vi "Network Close.vi"(8 "error in (no error)":errorcluster, 11 "Settings":T1={"UDP Receiver"=refnum, "UDP Sender"=refnum, "Valid Packet"=FALSE, "TCP"=refnum, "Network Settings"={"IP adress"="127.0.0.1", "RDB"={"Protocol"=enum."UDP", "Tx Port"=48270, "Rx Port"=10, "Buffer Size"=204800, "Timeout"=10}, "SCP"={"Protocol"=enum."TCP", "Tx Port"=48191, "Rx Port"=48191, "Buffer Size"=204800, "Timeout"=10}}, "vclient"=path "", "paeseHandle"=0, "builderHandle"=0}) -> (0 "error out":errorcluster)   [LabVIEW 2023, in "Vires VTD Engine.lvlib"]
uses:
  Vires VTD Engine.lvlib
  Type/Settings.ctl
  Shared/Network Settings.ctl
  Shared/Protocol.ctl
  Shared/Vires VTD Shared.lvlib
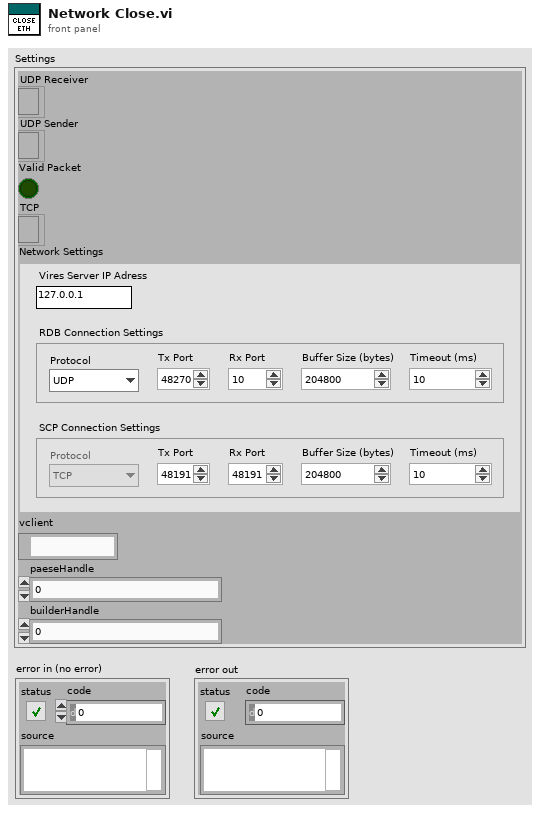
[diagram p1: front panel]
types:
  T1 = typedef "Vires VTD Engine.lvlib/Settings.ctl" = cluster{"UDP Receiver":refnum<k16>, "UDP Sender":refnum<k16>, "Valid Packet":bool, "TCP":refnum<k5>, "Network Settings":T2, "vclient":path, "paeseHandle":u64, "builderHandle":u64}
  T2 = typedef "Vires VTD Shared.lvlib/Network Settings.ctl" = cluster{"IP adress":string, "RDB":cluster{"Protocol":T3, "Tx Port":u16, "Rx Port":u16, "Buffer Size":i32, "Timeout":u16}, "SCP":cluster{"Protocol":T3, "Tx Port":u16, "Rx Port":u16, "Buffer Size":i32, "Timeout":u16}}
  T3 = typedef "Vires VTD Shared.lvlib/Protocol.ctl" = enum16{"UDP", "TCP"}
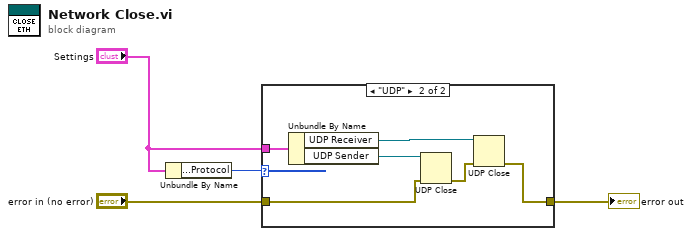
[diagram p0: block diagram]
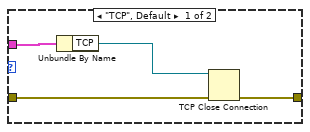
[diagram p2: hidden frame]
diagram:
  n1 = Unbundle By Name("Settings") -> ("Network Settings.RDB.Protocol"=w3:T3)
  n2 = case shown="\"UDP\"" w3 {
    tunnel: [w8 w14] -> w4
    tunnel: "Settings" -> [w6 w12]
    tunnel: "error in (no error)" -> [w7 w9]
    frame "TCP", Default {
      n3 = Unbundle By Name(w6) -> ("TCP"=w5:refnum<k5>)
      n4 = TCP Close Connection(connection ID=w5, error in (no error)=w7) -> (error out=w8:errorcluster)  [unwired: 1 in, 1 out]
    }
    frame "UDP" {
      n5 = Unbundle By Name(w12) -> ("UDP Receiver"=w11:refnum<k16>, "UDP Sender"=w10:refnum<k16>)
      n6 = UDP Close(connection ID=w10, 8:w9) -> (error out=w13:errorcluster)  [unwired: 1 out]
      n7 = UDP Close(connection ID=w11, 8:w13) -> (error out=w14:errorcluster)  [unwired: 1 out]
    }
  }
  "error out" <- w4
